vi "Configure.vi"(5 "Results Folder":path, 7 "Stopped Notification":refnum<notifier>, 8 "error in":errorcluster, 9 "Step Index Display":refnum<vi>, 10 "Status Display":refnum<vi>, 11 "Sequence Executor in":refnum<class "Sequence Executor.lvclass">) -> (0 "error out":errorcluster, 3 "Sequence Executor out":refnum<class "Sequence Executor.lvclass">)   [LabVIEW 2026, in "Sequence Executor.lvclass"]
doc: "Stores the Status Display, Step Index Display, Stopped Notification and Results Folder in the actor's private data. Called by the launcher BEFORE Launch Root Actor. Static, public. The remaining display refs are stored by Configure Displays.vi (pane 4815 has only 12 slots)."
uses:
  C:/Users/DynaAdmin/PycharmProjects/Universal-sequence-executor-AF/src/Executor/Sequence Executor.lvclass
  C:/Users/DynaAdmin/PycharmProjects/Universal-sequence-executor-AF/src/Executor/Sequence Executor.lvclass/Sequence Executor.ctl
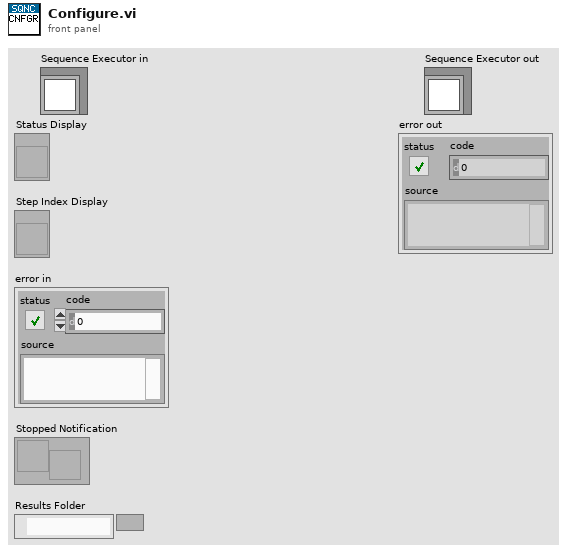
[diagram p1: front panel]
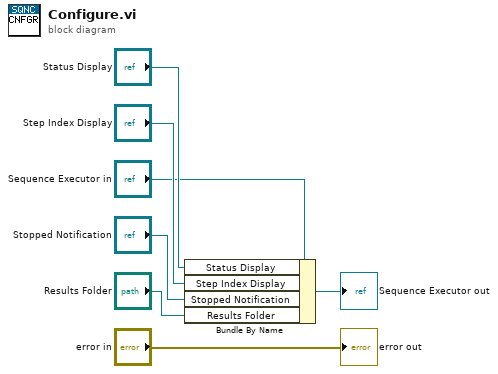
[diagram p0: block diagram]
diagram:
  n1 = Bundle By Name(cluster="Sequence Executor in", "Status Display"="Status Display", "Step Index Display"="Step Index Display", "Stopped Notification"="Stopped Notification", "Results Folder"="Results Folder") -> (→"Sequence Executor out":refnum<class "Sequence Executor.lvclass">)
  "error out" <- "error in"
